vi "WHILE.vi"() -> ()   [LabVIEW 2026]
panel:
  out "VECES":i16
  out "NUMERO ESPERADO: 6":dbl
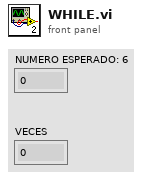
[diagram p1: front panel]
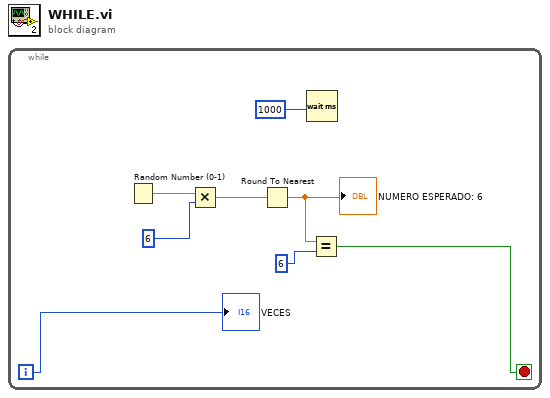
[diagram p0: block diagram]
diagram:
  n1 = while {
    i -> [w1]
    stop <- w3 stop-if-true
    n2 = Random Number (0-1)() -> (number: 0 to 1=w8:dbl)
    n3 = Multiply(x=w8, y=6) -> (x*y=w6:dbl)
    n4 = Round To Nearest(number=w6) -> (nearest integer value=w4:dbl)
    "NUMERO ESPERADO: 6" <- w4
    n5 = Wait (ms)(milliseconds to wait=1000) -> ()  [unwired: 1 out]
    n6 = Equal?(x=w4, y=6) -> (x = y?=w3:bool)
    "VECES" <- w1
  }
